vi "Event ElapsedTime.vi"(8 "error in (no error)":errorcluster, 10 "End in":refnum<class "Event.lvclass">, 11 "Start in":refnum<class "Event.lvclass">) -> (0 "error out":errorcluster, 1 "ElapsedTime [ms]":sgl, 2 "End out":refnum<class "Event.lvclass">, 3 "start out":refnum<class "Event.lvclass">)   [LabVIEW 2020, in "OpenLvVision_OpenCv.lvlib" / "Cuda.lvlib" / "Event.lvclass"]
doc: "Calculates the precise GPU execution time that elapsed between two recorded events."
uses:
  Event.lvclass
  C:/Users/lukas/Documents/OpenLvVision_OpenCv/SourceCode/LabView/OpenLvVision_OpenCv/_LvHelpers/EdvrObject/EdvrObject.lvclass
  _LvHelpers/EdvrObject/EdvrObject.lvclass/EdvrObject.ctl
  OpenLvVision_OpenCv.lvlib
  _LvHelpers/EdvrObject/EdvrObject.lvclass
  <vilib>/Utility/error.llb/Error Cluster From Error Code.vi
  <vilib>/ErrorRing/Error Ring.xnode
  Dlls/OlvOpenCvWrapper.dll
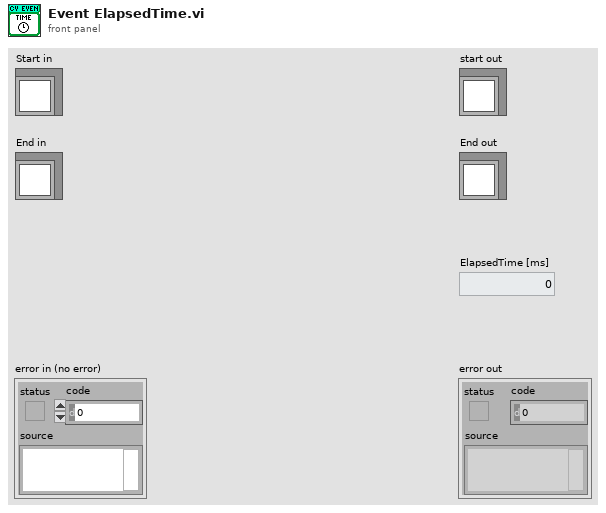
[diagram p1: front panel]
types:
  T1 = typedef "OpenLvVision_OpenCv.lvlib/EdvrObject.lvclass/Edvr.ctl" = refnum<data-value>
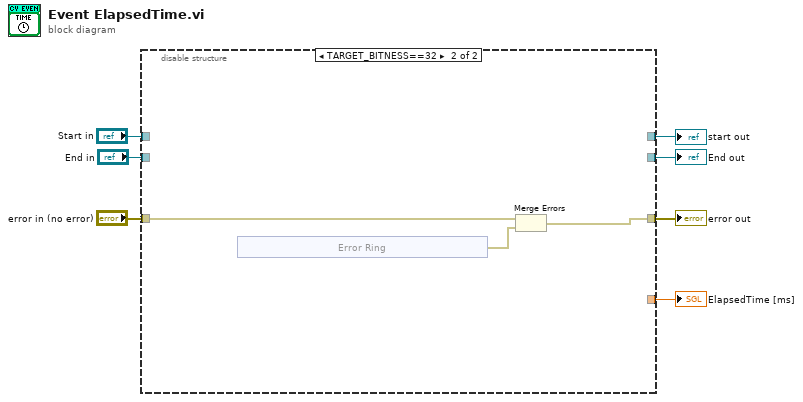
[diagram p0: block diagram]
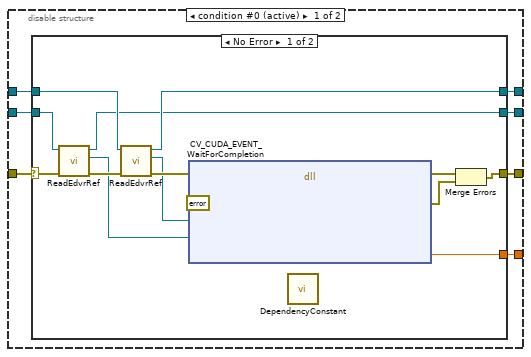
[diagram p2: hidden frame]
diagram:
  n1 = disable-structure shown="TARGET_BITNESS==32" {
    disable-tunnel: "error in (no error)" -> [w11 w33]
    disable-tunnel: [w14 w34] -> w7
    disable-tunnel: [w13 _] -> w6
    disable-tunnel: "Start in" -> [w12 _]
    disable-tunnel: "End in" -> [w10 _]
    disable-tunnel: [w9 _] -> w2
    disable-tunnel: [w8 _] -> w1
    frame condition #0 (active) {
      n2 = case shown="No Error" w11 {
        selector: w11 -> [w18 w31]
        tunnel: [w24 w31] -> w14
        tunnel: [w25 w30] -> w13
        tunnel: w12 -> [w23 w30]
        tunnel: w10 -> [w17 w29]
        tunnel: [w20 _] -> w9
        tunnel: [w16 w29] -> w8
        frame No Error {
          n3 = call "ReadEdvrRef.vi"("error in (no error)"=w18, "EdvrObject in"=w17) -> ("error out"=w19:errorcluster, "Edvr"=w15:T1, "EdvrObject out"=w16:refnum<class "Event.lvclass">)  [unwired: 7 in]
          n4 = call "ReadEdvrRef.vi"("error in (no error)"=w19, "EdvrObject in"=w23) -> ("error out"=w27:errorcluster, "Edvr"=w26:T1, "EdvrObject out"=w25:refnum<class "Event.lvclass">)  [unwired: 7 in]
          n5 = dll-call lib="C:/Users/lukas/Documents/OpenLvVision_OpenCv/SourceCode/LabView/OpenLvVision_OpenCv/Dlls/OlvOpenCvWrapper.dll" fn="CV_CUDA_EVENT_WaitForCompletion"(error in=w27, "Error"=errorcluster {"status"=FALSE, "code"=0, "source"=""} ("error out"), "startEdvrRef"=w26, "endEdvrRef"=w15) -> (error out=w21:errorcluster, "Error"=w22:errorcluster, "elapsedMs"=w20:sgl)  [unwired: 6 in, 1 out]
          n6 = call "DependencyConstant.vi"() -> ()  [unwired: 12 in]
          n7 = Merge Errors(w21, w22) -> (w24:errorcluster)
        }
        frame Error {
        }
      }
    }
    frame condition #1 {
      n8 = xnode "Error Ring"() -> ("error out"=w32:errorcluster)
      n9 = Merge Errors(w33, w32) -> (w34:errorcluster)
    }
  }
  "error out" <- w7
  "start out" <- w6
  "ElapsedTime [ms]" <- w2
  "End out" <- w1
